vi "ZMQ.Reconnect.vi"(8 "error in (no error)":errorcluster, 11 "RemoteControl.ZMQ in":refnum<class "RemoteControl.ZMQ.lvclass">) -> (0 "error out":errorcluster, 3 "RemoteControl.ZMQ out":refnum<class "RemoteControl.ZMQ.lvclass">)   [LabVIEW 2019, in "RemoteControl.ZMQ.lvlib" / "RemoteControl.ZMQ.lvclass"]
uses:
  RemoteControl.ZMQ.lvclass
  RemoteControl.ZMQ.lvclass/RemoteControl.ZMQ.ctl
  <vilib>/addons/zeromq/zeromq.lvlib
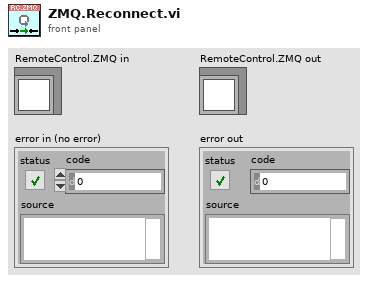
[diagram p1: front panel]
types:
  T1 = typedef "zeromq.lvlib/socket_type.ctl" = enum8{"ZMQ_PAIR", "ZMQ_PUB", "ZMQ_SUB", "ZMQ_REQ", "ZMQ_REP", "ZMQ_DEALER", "ZMQ_ROUTER", "ZMQ_PULL", "ZMQ_PUSH", "ZMQ_XPUB", "ZMQ_XSUB", "ZMQ_STREAM", "ZMQ_SERVER", "ZMQ_CLIENT", "ZMQ_RADIO", "ZMQ_DISH", "ZMQ_GATHER", "ZMQ_SCATTER", "ZMQ_DGRAM"}
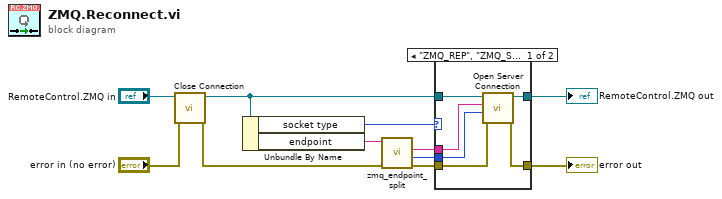
[diagram p0: block diagram]
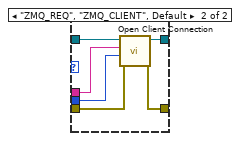
[diagram p2: hidden frame]
diagram:
  n1 = call-dynamic "Close Connection.vi"("error in (no error)"="error in (no error)", "RemoteControl.ZMQ in"="RemoteControl.ZMQ in") -> ("error out"=w3:errorcluster, "RemoteControl.ZMQ out"=w2:refnum<class "RemoteControl.ZMQ.lvclass">)  [unwired: 8 in]
  n2 = Unbundle By Name(w2) -> ("socket type"=w5:T1, "endpoint"=w8:string)
  n3 = call <vilib>:"zmq_endpoint_split.vi"("error in"=w3, "endpoint"=w8) -> ("error out"=w10:errorcluster, "port"=w6:u16, "address"=w7:string)  [unwired: 2 in, 1 out]
  n4 = case shown="\"ZMQ_REP\", \"ZMQ_SERVER\"" w5 {
    tunnel: w2 -> [w17 w23]
    tunnel: [w16 w22] -> w9
    tunnel: w6 -> [w14 w21]
    tunnel: w7 -> [w15 w20]
    tunnel: w10 -> [w13 w19]
    tunnel: [w12 w18] -> w11
    frame "ZMQ_REP", "ZMQ_SERVER" {
      n5 = call-dynamic "Open Server Connection.vi"("error in (no error)"=w13, "port"=w14, "address"=w15, "RemoteControl.ZMQ in"=w17) -> ("error out"=w12:errorcluster, "RemoteControl.ZMQ out"=w16:refnum<class "RemoteControl.ZMQ.lvclass">)  [unwired: 6 in]
    }
    frame "ZMQ_REQ", "ZMQ_CLIENT", Default {
      n6 = call-dynamic "Open Client Connection.vi"("error in (no error)"=w19, "port"=w21, "address"=w20, "RemoteControl.ZMQ in"=w23) -> ("error out"=w18:errorcluster, "RemoteControl.ZMQ out"=w22:refnum<class "RemoteControl.ZMQ.lvclass">)  [unwired: 6 in]
    }
  }
  "error out" <- w11
  "RemoteControl.ZMQ out" <- w9
